vi "Two Way Event Recorder Main Page.vi"(8 "error in (no error)":errorcluster, 11 "Node Ptr":T1 format="%.0x") -> (0 "error out":errorcluster)   [LabVIEW 2017, in "Two Way Event Recorder Custom Device.lvlib"]
uses:
  Two Way Event Recorder Custom Device.lvlib
  <vilib>/NI Veristand/Custom Device API/Custom Device Item Ref.ctl
  Two Way Event Recorder Property Lookup.vi
  <vilib>/NI Veristand/Custom Device API/Get Item Property (U16).vi
  <vilib>/NI Veristand/Custom Device API/Get Item Property (String).vi
  <vilib>/NI Veristand/Custom Device API/Get Item Property (U32).vi
  <vilib>/NI Veristand/Custom Device API/Set Item Property (U16).vi
  <vilib>/NI Veristand/Custom Device API/Set Item Property (String).vi
  <vilib>/NI Veristand/Custom Device API/Set Item Property (U32).vi
  <vilib>/NI VeriStand/Custom Device API/Custom Device API.lvlib
panel:
  in  "Timeout (mS)":u32
  in  "Flow Control":u16(ring) items=["None", "XON/XOFF", "RTS/CTS", "XON/XOFF & RTS/CTS", "DTR/DSR", "XON/XOFF & DTR/DSR"]
  in  "Stop Bits":u16(ring)=10 items=["1.0"=10, "1.5"=15, "2.0"=20]
  in  "Parity":u16(ring) items=["None", "Odd", "Even", "Mark", "Space"]
  in  "Data Bits":u16
  in  "Baud Rate":u32
  in  "Visa Ref":string
  in  "Start Bit":u16
  in  "Header":cluster{"Section Name":string}={"Section Name"="Custom Device Item Settings"}
  in  "Description":string
  in  "Name":string
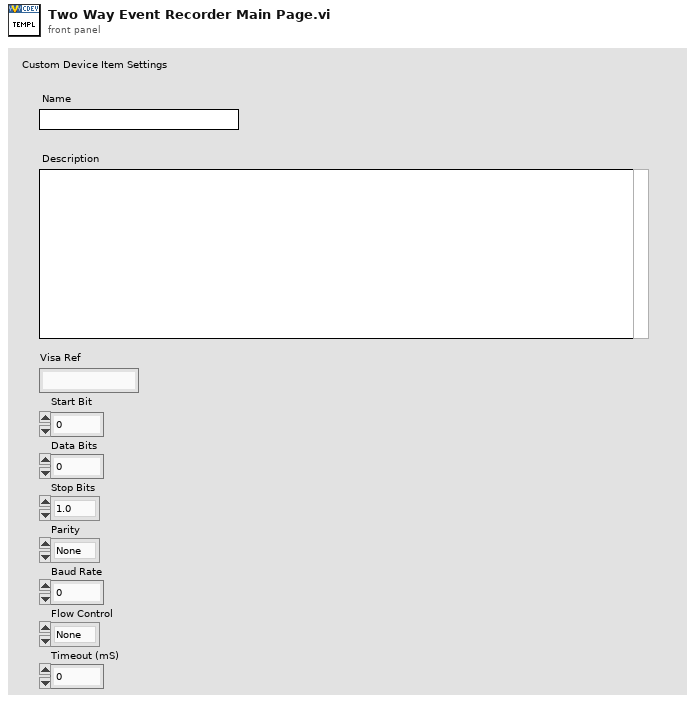
[diagram p1: front panel]
types:
  T1 = typedef "Custom Device API.lvlib/Custom Device Item Ref.ctl" = u64
  T2 = typedef "Custom Device API.lvlib/Custom Device Item Info.ctl" = cluster{"Name":string, "Is Channel":bool, "GUID":string, "Is Waveform":bool}
  T3 = typedef "Custom Device API.lvlib/Custom Device Commands.ctl" = enum16{"Default", "Item renamed", "Shutdown", "Dynamic button pressed"}
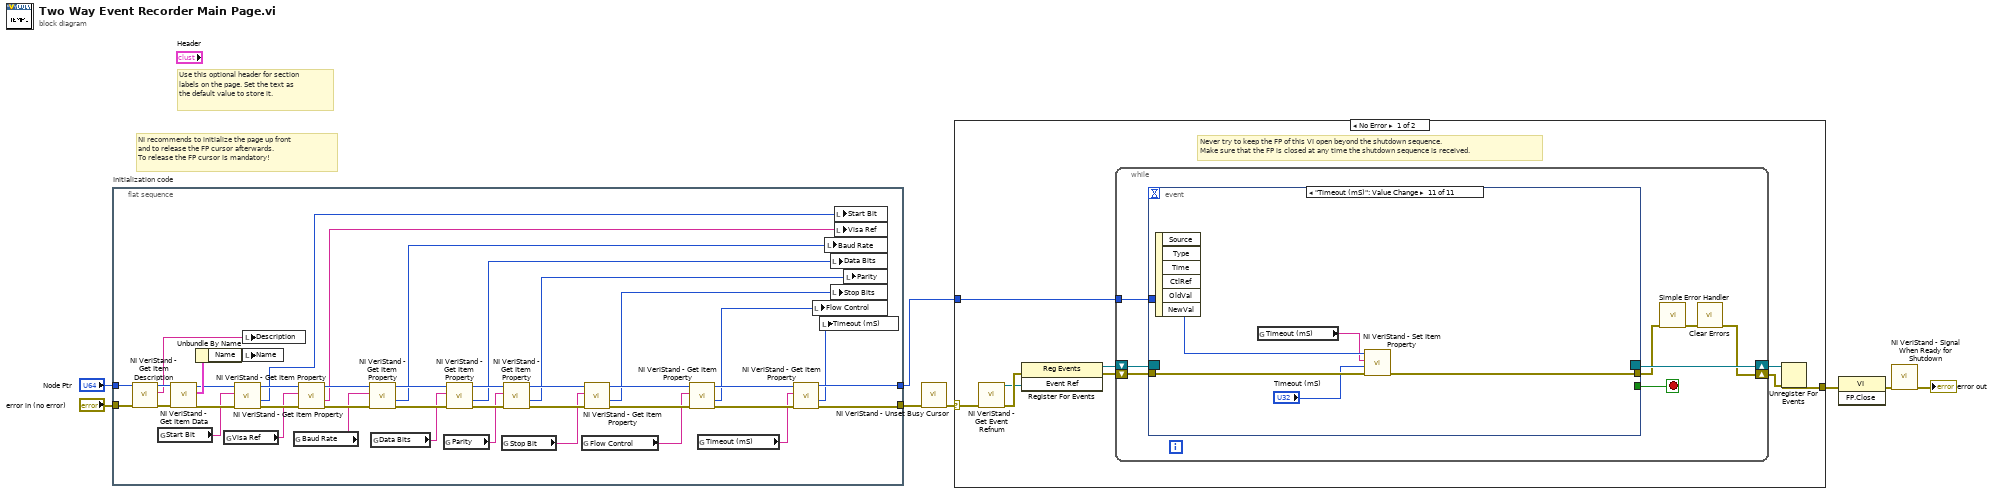
[diagram p0: block diagram]
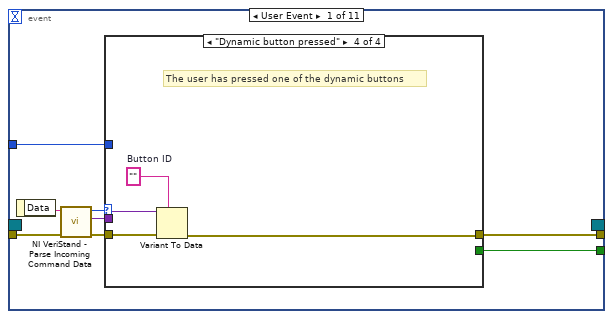
[diagram p2: hidden frame]
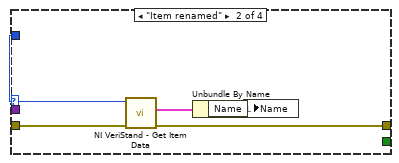
[diagram p4: hidden frame]
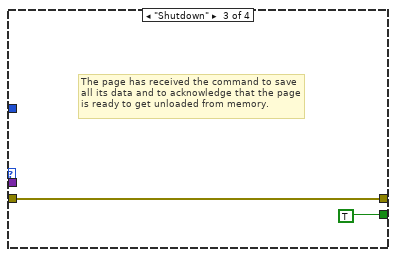
[diagram p5: hidden frame]
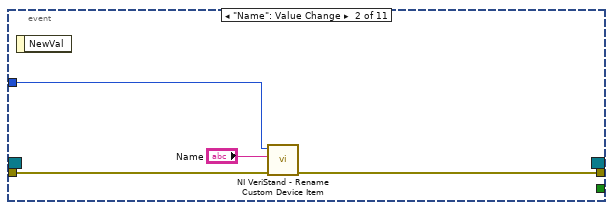
[diagram p6: hidden frame]
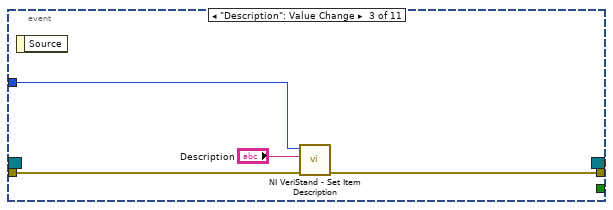
[diagram p7: hidden frame]
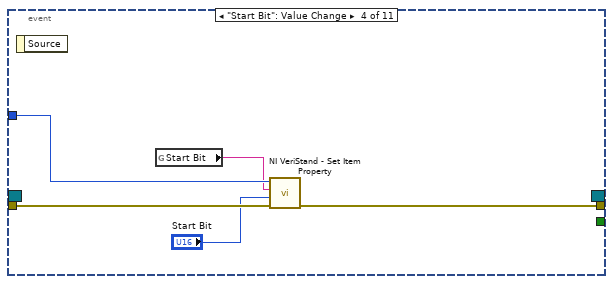
[diagram p8: hidden frame]
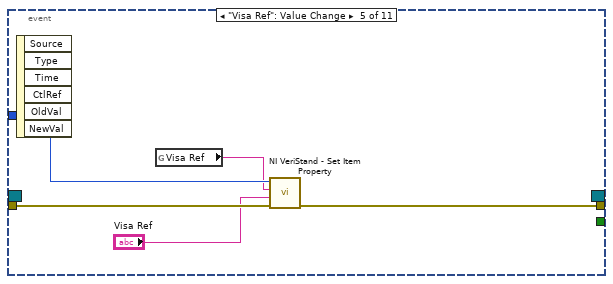
[diagram p9: hidden frame]
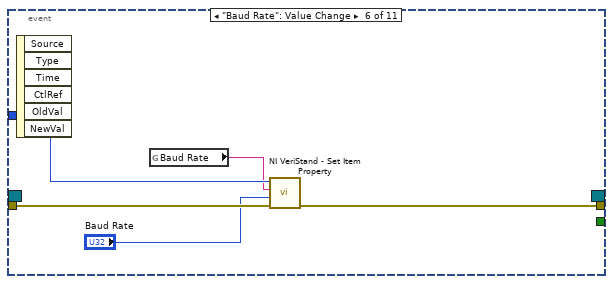
[diagram p10: hidden frame]
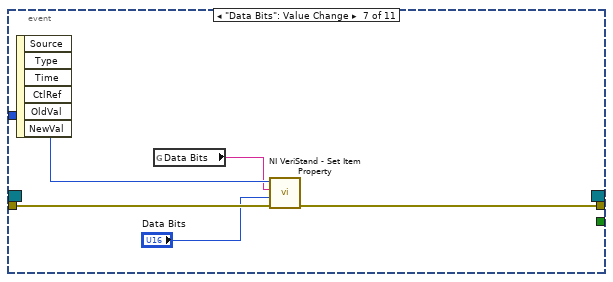
[diagram p11: hidden frame]
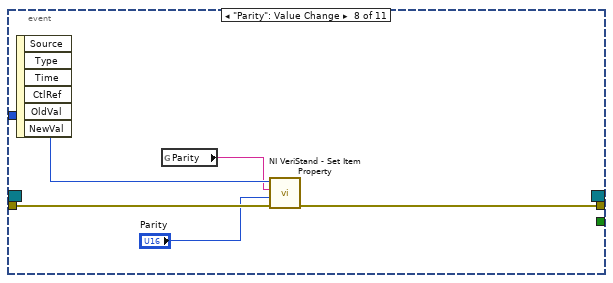
[diagram p12: hidden frame]
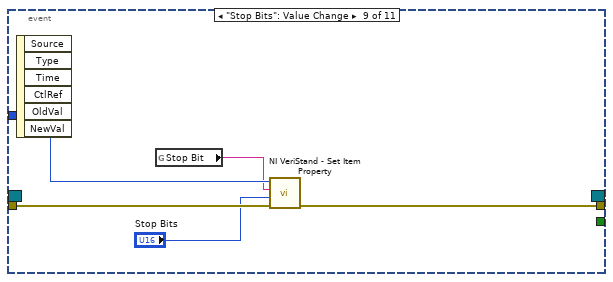
[diagram p13: hidden frame]
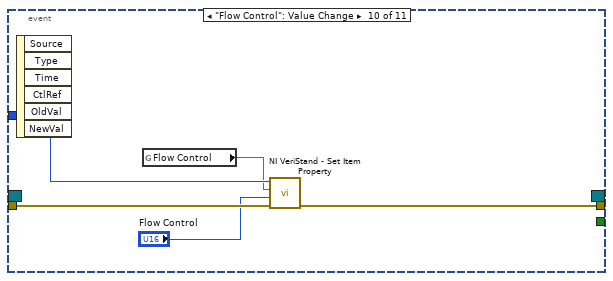
[diagram p14: hidden frame]
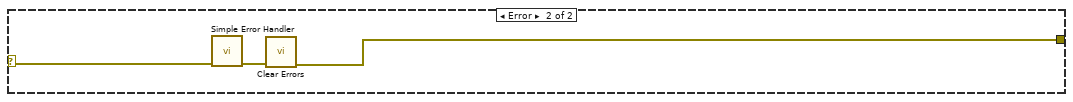
[diagram p15: hidden frame]
diagram:
  # "Use this optional header for section labels on the page. Set the text as the default value to store it."
  # "NI recommends to initialize the page up front\nand to release the FP cursor afterwards.\nTo release the FP cursor is mandatory!"
  n1 = flat-sequence "Initialization code" {
    tunnel: "error in (no error)" -> [w39]
    tunnel: "Node Ptr" -> [w38]
    tunnel: [w9] -> w4
    tunnel: [w49] -> w1
    frame #0 {
      n2 = call <vilib>:"NI VeriStand - Get Item Description.vi"("error in (no error)"=w39, "Item Ref in"=w38) -> ("error out"=w36:errorcluster, "Description"=w37:string, "Item Ref out"=w40:T1)  [unwired: 7 out]
      n3 = global read "Two Way Event Recorder Property Lookup.vi" "Start Bit"() -> (w31:string)
      n4 = call <vilib>:"NI VeriStand - Get Item Data.vi"("error in (no error)"=w36, "Item Ref in"=w40) -> ("error out"=w33:errorcluster, "Item Info"=w35:T2, "Item Ref out"=w32:T1)  [unwired: 7 out]
      n5 = Unbundle By Name(w35) -> ("Name"=w34:string)
      n6 = global read "Two Way Event Recorder Property Lookup.vi" "Visa Ref"() -> (w28:string)
      n7 = call-poly <vilib>:"NI VeriStand - Get Item Property.vi"("error in (no error)"=w33, "Property Name"=w31, "Item Ref in"=w32) -> ("error out"=w30:errorcluster, "Value"=w27:u16, "Item Ref out"=w29:T1)  [unwired: 5 in, 1 out]
      n8 = local write "Description"(w37) -> ()
      n9 = local write "Name"(w34) -> ()
      n10 = global read "Two Way Event Recorder Property Lookup.vi" "Baud Rate"() -> (w25:string)
      n11 = call-poly <vilib>:"NI VeriStand - Get Item Property.vi"("error in (no error)"=w30, "Property Name"=w28, "Item Ref in"=w29) -> ("error out"=w41:errorcluster, "Value"=w26:string, "Item Ref out"=w42:T1)  [unwired: 5 in, 1 out]
      n12 = call-poly <vilib>:"NI VeriStand - Get Item Property.vi"("error in (no error)"=w41, "Property Name"=w25, "Item Ref in"=w42) -> ("error out"=w23:errorcluster, "Value"=w24:u32, "Item Ref out"=w43:T1)  [unwired: 5 in, 1 out]
      n13 = global read "Two Way Event Recorder Property Lookup.vi" "Data Bits"() -> (w22:string)
      n14 = global read "Two Way Event Recorder Property Lookup.vi" "Parity"() -> (w19:string)
      n15 = call-poly <vilib>:"NI VeriStand - Get Item Property.vi"("error in (no error)"=w23, "Property Name"=w22, "Item Ref in"=w43) -> ("error out"=w20:errorcluster, "Value"=w21:u16, "Item Ref out"=w44:T1)  [unwired: 5 in, 1 out]
      n16 = global read "Two Way Event Recorder Property Lookup.vi" "Stop Bit"() -> (w16:string)
      n17 = call-poly <vilib>:"NI VeriStand - Get Item Property.vi"("error in (no error)"=w20, "Property Name"=w19, "Item Ref in"=w44) -> ("error out"=w17:errorcluster, "Value"=w18:u16, "Item Ref out"=w45:T1)  [unwired: 5 in, 1 out]
      n18 = global read "Two Way Event Recorder Property Lookup.vi" "Flow Control"() -> (w13:string)
      n19 = call-poly <vilib>:"NI VeriStand - Get Item Property.vi"("error in (no error)"=w17, "Property Name"=w16, "Item Ref in"=w45) -> ("error out"=w14:errorcluster, "Value"=w15:u16, "Item Ref out"=w46:T1)  [unwired: 5 in, 1 out]
      n20 = call-poly <vilib>:"NI VeriStand - Get Item Property.vi"("error in (no error)"=w14, "Property Name"=w13, "Item Ref in"=w46) -> ("error out"=w47:errorcluster, "Value"=w12:u16, "Item Ref out"=w48:T1)  [unwired: 5 in, 1 out]
      n21 = global read "Two Way Event Recorder Property Lookup.vi" "Timeout (mS)"() -> (w11:string)
      n22 = call-poly <vilib>:"NI VeriStand - Get Item Property.vi"("error in (no error)"=w47, "Property Name"=w11, "Item Ref in"=w48) -> ("error out"=w9:errorcluster, "Value"=w10:u32, "Item Ref out"=w49:T1)  [unwired: 5 in, 1 out]
      n23 = local write "Flow Control"(w12) -> ()
      n24 = local write "Timeout (mS)"(w10) -> ()
      n25 = local write "Baud Rate"(w24) -> ()
      n26 = local write "Data Bits"(w21) -> ()
      n27 = local write "Stop Bits"(w15) -> ()
      n28 = local write "Start Bit"(w27) -> ()
      n29 = local write "Visa Ref"(w26) -> ()
      n30 = local write "Parity"(w18) -> ()
    }
  }
  n31 = call <vilib>:"NI VeriStand - Unset Busy Cursor.vi"("error in (no error)"=w4) -> ("error out"=w3:errorcluster)  [unwired: 10 out]
  n32 = case shown="No Error" w3 {
    selector: w3 -> [w50 w137]
    tunnel: [w55 w135] -> w8
    tunnel: w1 -> [w51 _]
    frame No Error {
      # "Never try to keep the FP of this VI open beyond the shutdown sequence.\nMake sure that the FP is closed at any time the shutdown sequence is received."
      n33 = call <vilib>:"NI VeriStand - Get Event Refnum.vi"("error in (no error)"=w50) -> ("error out"=w58:errorcluster, "Event Ref"=w54:refnum<user-event>)  [unwired: 9 out]
      n34 = register-events(error in=w58, w54) -> (reference out=w52:refnum<event-registration>, error out=w53:errorcluster)  [unwired: 1 in]
      n35 = while {
        tunnel: w51 -> [w62]
        shift-right: [w59] -> w56
        shift-left: w53 -> [w65]
        shift-right: [w66] -> w57
        shift-left: w52 -> [w64]
        stop <- w63 stop-if-true
        n36 = event shown="[10] \"Timeout (mS)\": Value Change" {
          selector: w64 -> [_ _ _ _ _ _ _ _ _ _ _]
          dyn-events: [_ _ _ _ _ _ _ _ _ _ _] -> w66
          timeout: _ -> [_ _ _ _ _ _ _ _ _ _ _]
          tunnel: w65 -> [w74 w90 w93 w99 w104 w109 w114 w119 w124 w129 w134]
          tunnel: [w70 _ _ _ _ _ _ _ _ _ _] -> w63
          tunnel: [w69 w89 w92 w95 w101 w106 w111 w116 w121 w126 w131] -> w61
          tunnel: w62 -> [w68 w88 w94 w98 w103 w108 w113 w118 w123 w128 w133]
          event User Event {
            n37 = event-data() -> ("Data"=w73:string)  [unwired: 1 out]
            n38 = call <vilib>:"NI VeriStand - Parse Incoming Command Data.vi"("error in (no error)"=w74, "Incoming data"=w73) -> ("error out"=w72:errorcluster, "Outgoing data"=w67:variant, "Action"=w71:T3)  [unwired: 7 out]
            n39 = case shown="\"Dynamic button pressed\"" w71 {
              tunnel: w72 -> [w75 w80 w81 w86]
              tunnel: [_ _ TRUE _] -> w70
              tunnel: [w75 w77 w81 w83] -> w69
              tunnel: w68 -> [_ w79 _ _]
              tunnel: w67 -> [_ _ _ w85]
              frame "Default", Default {
              }
              frame "Item renamed" {
                n40 = call <vilib>:"NI VeriStand - Get Item Data.vi"("error in (no error)"=w80, "Item Ref in"=w79) -> ("error out"=w77:errorcluster, "Item Info"=w78:T2)  [unwired: 8 out]
                n41 = Unbundle By Name(w78) -> ("Name"=w76:string)
                n42 = local write "Name"(w76) -> ()
              }
              frame "Shutdown" {
                # "The page has received the command to save all its data and to acknowledge that the page is ready to get unloaded from memory."
              }
              frame "Dynamic button pressed" {
                w84 = ""  # Button ID
                # "The user has pressed one of the dynamic buttons"
                n43 = Variant To Data(error in=w86, type=w84, Variant=w85) -> (error out=w83:errorcluster)  [unwired: 1 out]
              }
            }
          }
          event "Name": Value Change {
            n44 = event-data() -> ()  [unwired: 2 out]
            n45 = call <vilib>:"NI VeriStand - Rename Custom Device Item.vi"("error in (no error)"=w90, "New Name"="Name", "Item Ref in"=w88) -> ("error out"=w89:errorcluster)  [unwired: 1 in, 7 out]
          }
          event "Description": Value Change {
            n46 = event-data() -> ()  [unwired: 2 out]
            n47 = call <vilib>:"NI VeriStand - Set Item Description.vi"("error in (no error)"=w93, "Description"="Description", "Item Ref in"=w94) -> ("error out"=w92:errorcluster)  [unwired: 8 out]
          }
          event "Start Bit": Value Change {
            n48 = event-data() -> ()  [unwired: 2 out]
            n49 = global read "Two Way Event Recorder Property Lookup.vi" "Start Bit"() -> (w96:string)
            n50 = call-poly <vilib>:"NI VeriStand - Set Item Property.vi"("error in (no error)"=w99, "Value"="Start Bit", "Property Name"=w96, "Item Ref in"=w98) -> ("error out"=w95:errorcluster)  [unwired: 5 in, 2 out]
          }
          event "Visa Ref": Value Change {
            n51 = event-data() -> ()  [unwired: 7 out]
            n52 = global read "Two Way Event Recorder Property Lookup.vi" "Visa Ref"() -> (w102:string)
            n53 = call-poly <vilib>:"NI VeriStand - Set Item Property.vi"("error in (no error)"=w104, "Value"="Visa Ref", "Property Name"=w102, "Item Ref in"=w103) -> ("error out"=w101:errorcluster)  [unwired: 5 in, 2 out]
          }
          event "Baud Rate": Value Change {
            n54 = event-data() -> ()  [unwired: 7 out]
            n55 = global read "Two Way Event Recorder Property Lookup.vi" "Baud Rate"() -> (w107:string)
            n56 = call-poly <vilib>:"NI VeriStand - Set Item Property.vi"("error in (no error)"=w109, "Value"="Baud Rate", "Property Name"=w107, "Item Ref in"=w108) -> ("error out"=w106:errorcluster)  [unwired: 5 in, 2 out]
          }
          event "Data Bits": Value Change {
            n57 = event-data() -> ()  [unwired: 7 out]
            n58 = global read "Two Way Event Recorder Property Lookup.vi" "Data Bits"() -> (w112:string)
            n59 = call-poly <vilib>:"NI VeriStand - Set Item Property.vi"("error in (no error)"=w114, "Value"="Data Bits", "Property Name"=w112, "Item Ref in"=w113) -> ("error out"=w111:errorcluster)  [unwired: 5 in, 2 out]
          }
          event "Parity": Value Change {
            n60 = event-data() -> ()  [unwired: 7 out]
            n61 = global read "Two Way Event Recorder Property Lookup.vi" "Parity"() -> (w117:string)
            n62 = call-poly <vilib>:"NI VeriStand - Set Item Property.vi"("error in (no error)"=w119, "Value"="Parity", "Property Name"=w117, "Item Ref in"=w118) -> ("error out"=w116:errorcluster)  [unwired: 5 in, 2 out]
          }
          event "Stop Bits": Value Change {
            n63 = event-data() -> ()  [unwired: 7 out]
            n64 = global read "Two Way Event Recorder Property Lookup.vi" "Stop Bit"() -> (w122:string)
            n65 = call-poly <vilib>:"NI VeriStand - Set Item Property.vi"("error in (no error)"=w124, "Value"="Stop Bits", "Property Name"=w122, "Item Ref in"=w123) -> ("error out"=w121:errorcluster)  [unwired: 5 in, 2 out]
          }
          event "Flow Control": Value Change {
            n66 = event-data() -> ()  [unwired: 7 out]
            n67 = global read "Two Way Event Recorder Property Lookup.vi" "Flow Control"() -> (w127:string)
            n68 = call-poly <vilib>:"NI VeriStand - Set Item Property.vi"("error in (no error)"=w129, "Value"="Flow Control", "Property Name"=w127, "Item Ref in"=w128) -> ("error out"=w126:errorcluster)  [unwired: 5 in, 2 out]
          }
          event "Timeout (mS)": Value Change {
            n69 = event-data() -> ()  [unwired: 7 out]
            n70 = global read "Two Way Event Recorder Property Lookup.vi" "Timeout (mS)"() -> (w132:string)
            n71 = call-poly <vilib>:"NI VeriStand - Set Item Property.vi"("error in (no error)"=w134, "Value"="Timeout (mS)", "Property Name"=w132, "Item Ref in"=w133) -> ("error out"=w131:errorcluster)  [unwired: 5 in, 2 out]
          }
        }
        n72 = call <vilib>:"Simple Error Handler.vi"("error in (no error)"=w61) -> ("error out"=w60:errorcluster)  [unwired: 1 in, 7 out]
        n73 = call <vilib>:"Clear Errors.vi"("error in (no error)"=w60) -> ("error out"=w59:errorcluster)  [unwired: 1 in, 5 out]
      }
      n74 = Unregister For Events(event registration refnum=w57, error in=w56) -> (error out=w55:errorcluster)
    }
    frame Error {
      n75 = call <vilib>:"Simple Error Handler.vi"("error in (no error)"=w137) -> ("error out"=w136:errorcluster)  [unwired: 1 in, 7 out]
      n76 = call <vilib>:"Clear Errors.vi"("error in (no error)"=w136) -> ("error out"=w135:errorcluster)  [unwired: 1 in, 5 out]
    }
  }
  n77 = invoke class="VI" method="FP.Close"(error in=w8) -> (error out=w7:errorcluster)  [unwired: 2 in, 2 out]
  n78 = call <vilib>:"NI VeriStand - Signal When Ready for Shutdown.vi"("error in (no error)"=w7) -> ("error out"=→"error out":errorcluster)  [unwired: 10 out]
